vi "Data entry form.vi"(0 "Stack in":refnum<class "Stack.lvclass">, 1 "Adhesive type":string, 2 "Temperature (C)":string, 3 "Relative humidity":string, 5 "Position":dbl, 7 "Module Type":string="CMU,LD,Full,200,CuW", 9 "Module?":bool, 11 "error in (no error)":errorcluster, 12 "Operator":string, 13 "ROC version":string) -> (4 "Stack out":refnum<class "Stack.lvclass">, 8 "Cancelled?":bool, 15 "error out":errorcluster)   [LabVIEW 2021, in "Stack.lvclass"]
uses:
  Stack.lvclass
  Stack.lvclass/Stack.ctl
panel:
  in  "Tape Batch (optional)":string
  out "Time":string
  in  "?":string="Scan module QR code for real runs. For dummy runs leave empty."
  in  "Module stack name (no hyphens; include 320)":string
  in  "Cancel Button":bool
  in  "Comments":string
  in  "?":string="Leave Base/Top Layer ID fields empty for dummy runs!!"
  in  "?":string="Record sensor visual inspection comments here."
  out "Sensor thickness":string
  out "BP Type":string
  out "Geometry":string
  in  "Baselayer thickness for glue dispense":dbl
  out "Resolution":string
  out "Date":string
  in  "Glue Batch":string
  in  "Component Tray ID":string
  in  "Assembly Tray ID":string
  in  "PUT ID":string
  in  "Baselayer ID":string
  in  "Toplayer ID":string
  in  "Submit":bool
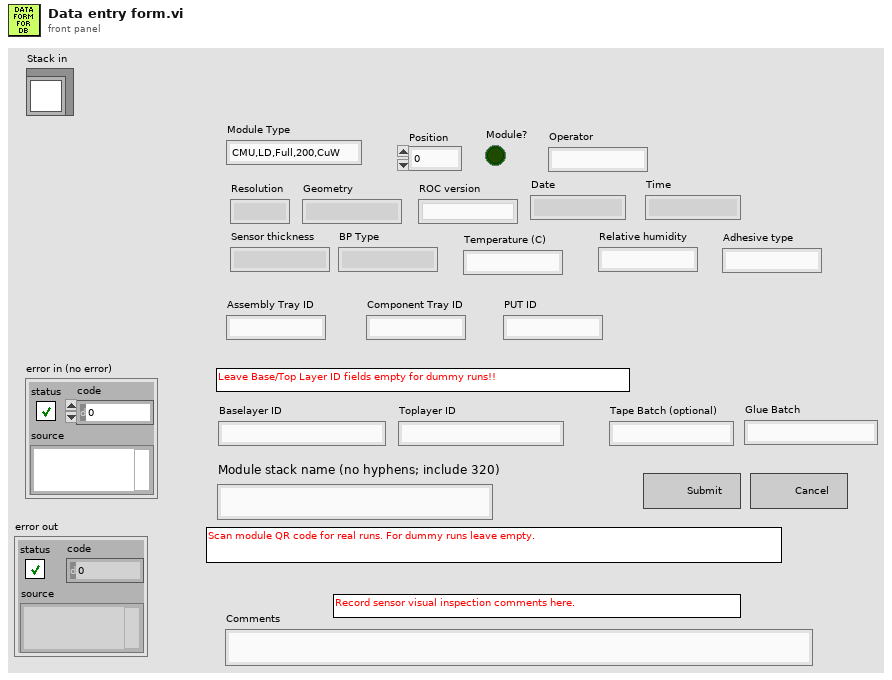
[diagram p1: front panel]
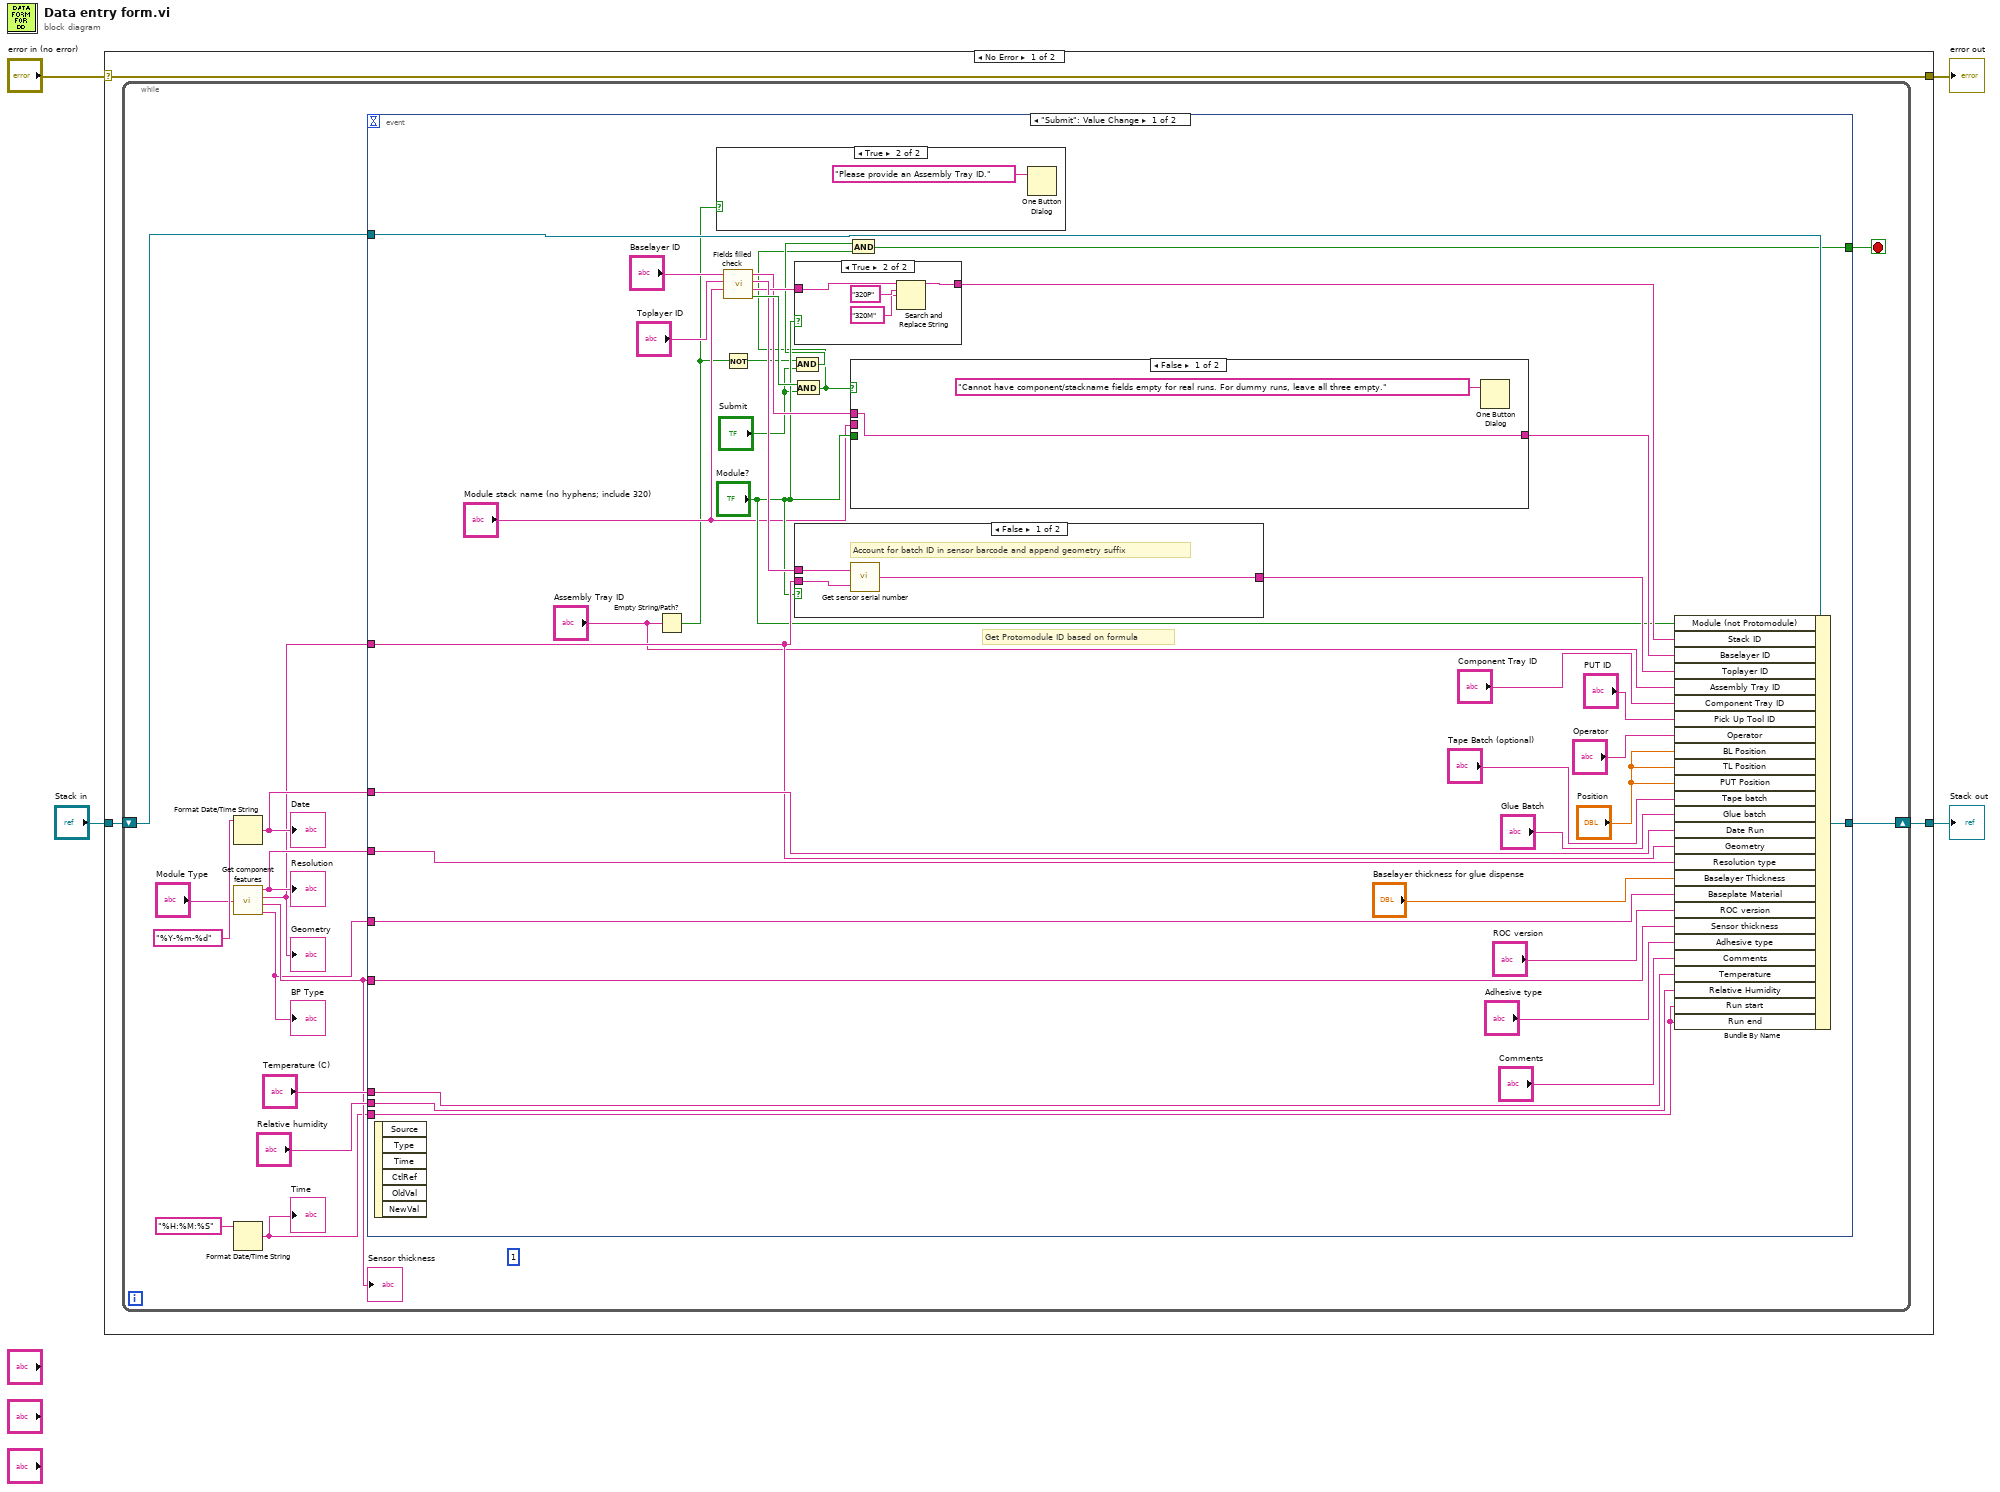
[diagram p0: block diagram]
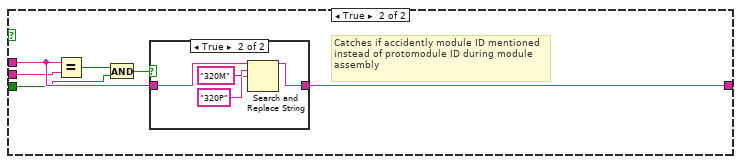
[diagram p3: hidden frame]
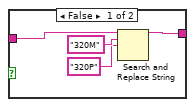
[diagram p5: hidden frame]
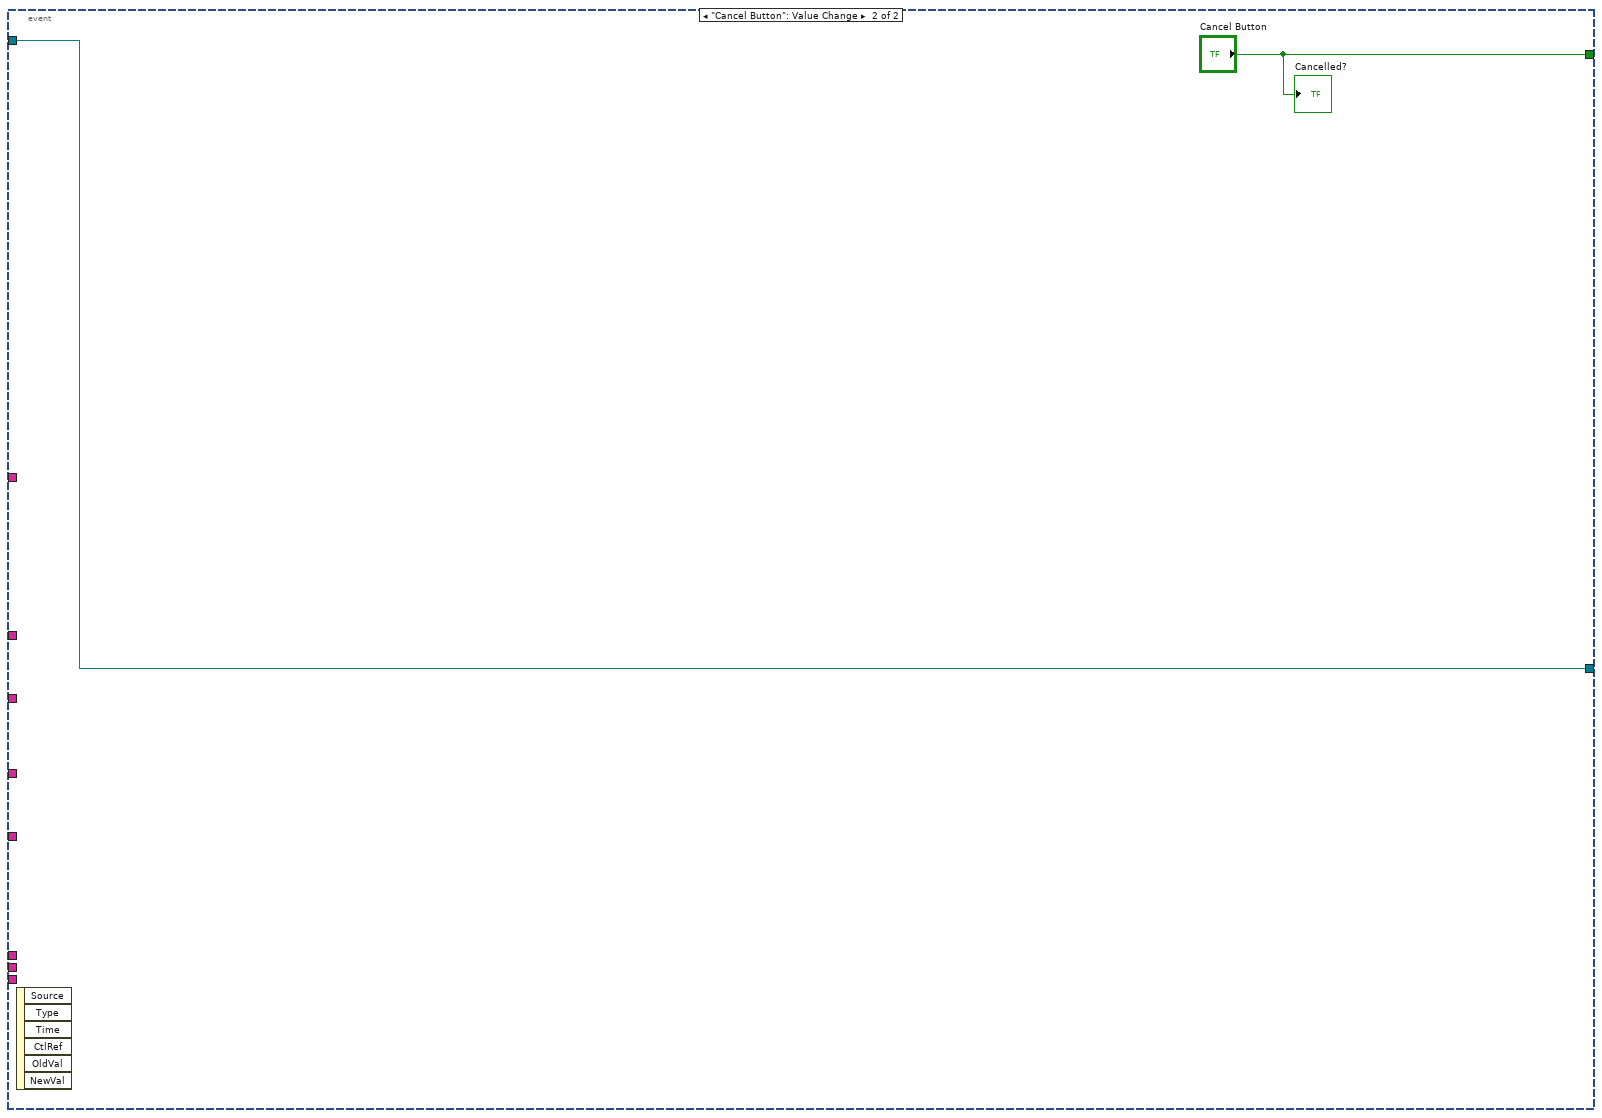
[diagram p7: hidden frame]
diagram:
  n1 = case shown="No Error" "error in (no error)" {
    selector: "error in (no error)" -> [w7 w89]
    tunnel: [w7 w89] -> w3
    tunnel: [w5 w88] -> w1
    tunnel: "Stack in" -> [w6 w88]
    frame No Error {
      n2 = while {
        shift-right: [w21] -> w5
        shift-left: w6 -> [w15]
        stop <- w16 stop-if-true
        (unwired) 1 ("offset (0)")
        n3 = Format Date/Time String(time format string (%c)="%Y-%m-%d") -> (date/time string=w19:string)  [unwired: 2 in]
        "Date" <- w19
        n4 = call "Get component features.vi"("Module Type"="Module Type") -> ("Resolution"=w13:string, "Geometry"=w12:string, "Sensor thickness"=w11:string, "BP Type"=w10:string)  [unwired: 1 in, 1 out]
        "Resolution" <- w13
        "Geometry" <- w12
        "BP Type" <- w10
        "Sensor thickness" <- w11
        n5 = Format Date/Time String(time format string (%c)="%H:%M:%S") -> (date/time string=w8:string)  [unwired: 2 in]
        "Time" <- w8
        n6 = event shown="[0] \"Submit\": Value Change" {
          selector: _ -> [_ _]
          dyn-events: _ -> [_ _]
          timeout: _ -> [_ _]
          tunnel: w15 -> [w59 w87]
          tunnel: [w55 w87] -> w21
          tunnel: w13 -> [w51 _]
          tunnel: w10 -> [w50 _]
          tunnel: w11 -> [w49 _]
          tunnel: w19 -> [w48 _]
          tunnel: w12 -> [w38 _]
          tunnel: "Temperature (C)" -> [w46 _]
          tunnel: "Relative humidity" -> [w45 _]
          tunnel: [w22 "Cancel Button"] -> w16
          tunnel: w8 -> [w37 _]
          event "Submit": Value Change {
            # "Get Protomodule ID based on formula"
            n7 = event-data() -> ()  [unwired: 1 in, 6 out]
            n8 = Empty String/Path?(string/path="Assembly Tray ID") -> (empty?=w27:bool)
            n9 = case shown="True" w27 {
              frame False {
              }
              frame True {
                n10 = One Button Dialog(message="Please provide an Assembly Tray ID.") -> ()  [unwired: 1 in, 1 out]
              }
            }
            n11 = call "Fields filled check.vi"("Module stack name (no hyphens; include 320)"="Module stack name (no hyphens; include 320)", "Toplayer ID"="Toplayer ID", "Baselayer ID"="Baselayer ID") -> ("Fields fully (not)filled"=w41:bool, "Module stack name (no hyphens; include 320) out"=w39:string, "Toplayer ID out"=w40:string, "Baselayer ID  out"=w31:string)  [unwired: 1 in]
            n12 = Not(x=w27) -> (.not. x?=w26:bool)
            n13 = And(x=w26, y="Submit") -> (x .and. y?=w25:bool)
            n14 = And(x=w41, y="Submit") -> (x .and. y?=w23:bool)
            n15 = case shown="True" "Module?" {
              tunnel: w39 -> [w75 w79]
              tunnel: [w74 w78] -> w44
              frame False {
                n16 = Search and Replace String(input string=w75, search string="320M", replace string="320P" ("replace string (\"\")")) -> (result string=w74:string)  [unwired: 5 in, 3 out]
              }
              frame True {
                n17 = Search and Replace String(input string=w79, search string="320P", replace string="320M" ("replace string (\"\")")) -> (result string=w78:string)  [unwired: 5 in, 3 out]
              }
            }
            n18 = case shown="False" "Module?" {
              tunnel: w38 -> [w83 _]
              tunnel: w40 -> [w84 w85]
              tunnel: [w82 w85] -> w47
              frame False {
                # "Account for batch ID in sensor barcode and append geometry suffix"
                n19 = call "Get sensor serial number.vi"("Geometry"=w83, "Toplayer ID"=w84) -> ("Toplayer ID out"=w82:string)
              }
              frame True {
              }
            }
            n20 = And(x=w25, y=w23) -> (x .and. y?=w22:bool)
            n21 = case shown="False" w23 {
              tunnel: w31 -> [w61 w67]
              tunnel: [w61 w68] -> w30
              tunnel: "Module?" -> [_ w64]
              tunnel: "Module stack name (no hyphens; include 320)" -> [_ w66]
              frame False {
                n22 = One Button Dialog(message="Cannot have component/stackname fields empty for real runs. For dummy runs, leave all three empty.") -> ()  [unwired: 1 in, 1 out]
              }
              frame True {
                # "Catches if accidently module ID mentioned instead of protomodule ID during module assembly"
                n23 = Equal?(x=w67, y=w66) -> (x = y?=w65:bool)
                n24 = And(x=w65, y=w64) -> (x .and. y?=w63:bool)
                n25 = case shown="True" w63 {
                  tunnel: w67 -> [w69 w71]
                  tunnel: [w69 w70] -> w68
                  frame False {
                  }
                  frame True {
                    n26 = Search and Replace String(input string=w71, search string="320M", replace string="320P" ("replace string (\"\")")) -> (result string=w70:string)  [unwired: 5 in, 3 out]
                  }
                }
              }
            }
            n27 = Bundle By Name(cluster=w59, "Module (not Protomodule)"="Module?", "Stack ID"=w44, "Baselayer ID"=w30, "Toplayer ID"=w47, "Assembly Tray ID"="Assembly Tray ID", "Component Tray ID"="Component Tray ID", "Pick Up Tool ID"="PUT ID", "Operator"="Operator", "BL Position"="Position", "TL Position"="Position", "PUT Position"="Position", "Tape batch"="Tape Batch (optional)", "Glue batch"="Glue Batch", "Date Run"=w48, "Geometry"=w38, "Resolution type"=w51, "Baselayer Thickness"="Baselayer thickness for glue dispense", "Baseplate Material"=w50, "ROC version"="ROC version", "Sensor thickness"=w49, "Adhesive type"="Adhesive type", "Comments"="Comments", "Temperature"=w46, "Relative Humidity"=w45, "Run start"=w37, "Run end"=w37) -> (w55:refnum<class "Stack.lvclass">)
          }
          event "Cancel Button": Value Change {
            n28 = event-data() -> ()  [unwired: 1 in, 6 out]
            "Cancelled?" <- "Cancel Button"
          }
        }
      }
    }
    frame Error {
    }
  }
  "error out" <- w3
  "Stack out" <- w1
